vi "RemoteVI Service Client.vi"(0 "Client":T2, 1 "windows":T3(array[cluster]), 5 "geo":T4, 7 "hWnd":u64, 9 "popups":T1, 11 "error in":errorcluster) -> (4 "Client out":T2, 6 "clicked?":bool, 8 "popups out":T1, 15 "error out":errorcluster)   [LabVIEW 2020, in "RemoteVI.lvlib"]
doc: "Services one WebSocket client without blocking (docs\\protocol.md sections 4-6). Reads whatever bytes are waiting (TCP Read, immediate mode, timeout 0; error 56 means nothing waiting, any other error means the peer is gone and sets closed), appends them to rx buffer and decodes every complete frame with RemoteVI WS Decode Client Frame.vi. A text frame goes through RemoteVI Parse Input.vi: an ack raises acked to max(acked, seq) when seq is not ahead of the client's seq; mouse and key messages first update mods (RemoteVI Track Modifiers.vi) and, when they changed and no popup is open, write them into the key state of LabVIEW's UI thread (RemoteVI Apply Modifiers.vi - LabVIEW reads Shift/Ctrl/Alt with GetKeyState, which posted messages do not update), then are translated (RemoteVI Translate Input.vi with geo, popup = popups.windows not empty, and tracking in = LabVIEW holds the mouse capture, RemoteVI Mouse Captured.vi) and posted to the window hWnd (RemoteVI Post Input.vi, which - while a popup is open - moves the invisible popups so that the clicked point lies under the host cursor, never moving the cursor, and waits until the popups change, at most 300 ms; the displacement it used travels on to the next message and out in popups out); a minimized panel is restored first (RemoteVI Restore If Minimized.vi). No VI Server call, so servicing goes on while an open LabVIEW popup blocks the UI thread; the server loop supplies geo, hWnd and popups from its cache. clicked? tells the server loop that a message which may open a LabVIEW popup (anything but WM_MOUSEMOVE and WM_MOUSEWHEEL) was posted, so it holds its VI Server calls back until the popup has had time to appear. A ping is answered with a pong; a close frame with a close frame (1000); a binary or fragmented message with close 1008; a protocol violation with the decoder's close code - each sets closed. Consumed bytes leave rx buffer. A click on a popup is posted no sooner than 350 ms after the popup was first seen open (popup since): LabVIEW ignores a click on a ring menu that arrives within about 250 ms of opening it (measured with posted messages: 200 ms ignored, 250 ms chosen). A client that closes with modifiers written is released (mods set back to 0, unless a popup is open). Mouse and key messages go to the window RemoteVI Route Input.vi picks among windows (docs\\protocol.md section 7); key window - the window the client last pressed a button in - travels from message to message. A client already closed is passed through untouched. TCP errors only set closed; error out carries the errors of restoring the window and posting input."
uses:
  RemoteVI.lvlib
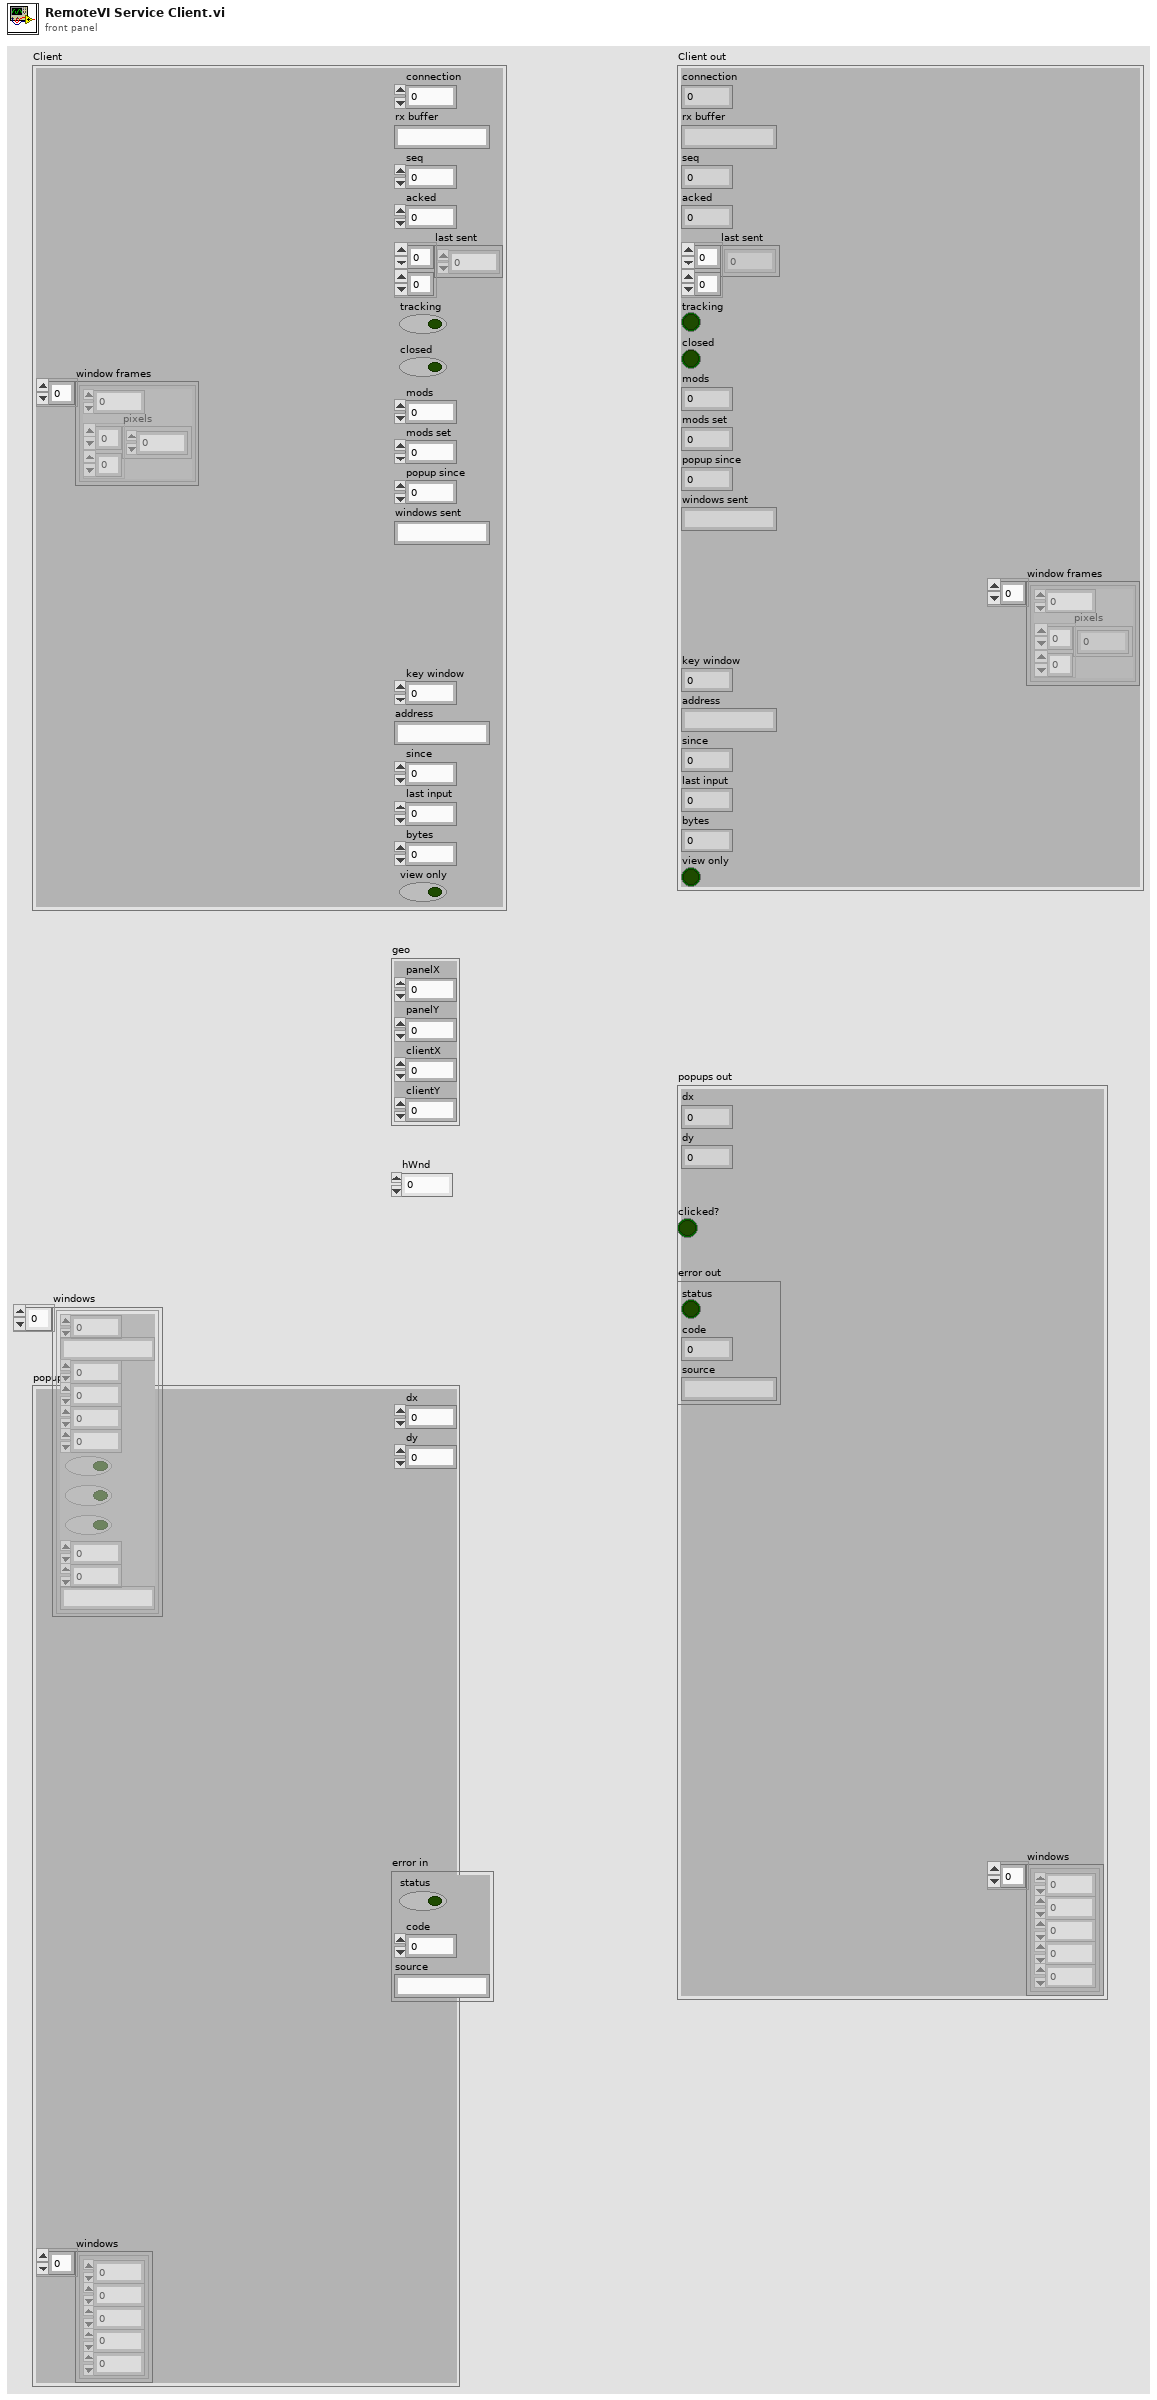
[diagram p1: front panel]
types:
  T1 = cluster{"windows":cluster{"hwnd":u64, "x":i32, "y":i32, "w":i32, "h":i32}[], "dx":i32, "dy":i32}
  T2 = cluster{"connection":u32, "rx buffer":string, "seq":u32, "acked":u32, "last sent":u32[][], "tracking":bool, "closed":bool, "mods":u8, "mods set":u8, "popup since":u32, "windows sent":string, "window frames":cluster{"id":u64, "pixels":u32[][]}[], "key window":u64, "address":string, "since":dbl, "last input":dbl, "bytes":dbl, "view only":bool}
  T3 = cluster{"id":u64, "title":string, "x":i32, "y":i32, "w":i32, "h":i32, "modal":bool, "active":bool, "closable":bool, "sx":i32, "sy":i32, "class":string}[]
  T4 = cluster{"panelX":i32, "panelY":i32, "clientX":i32, "clientY":i32}
  T5 = cluster{"hWnd":u64, "popup":bool, "geo":cluster{"panelX":i32, "panelY":i32, "clientX":i32, "clientY":i32}}
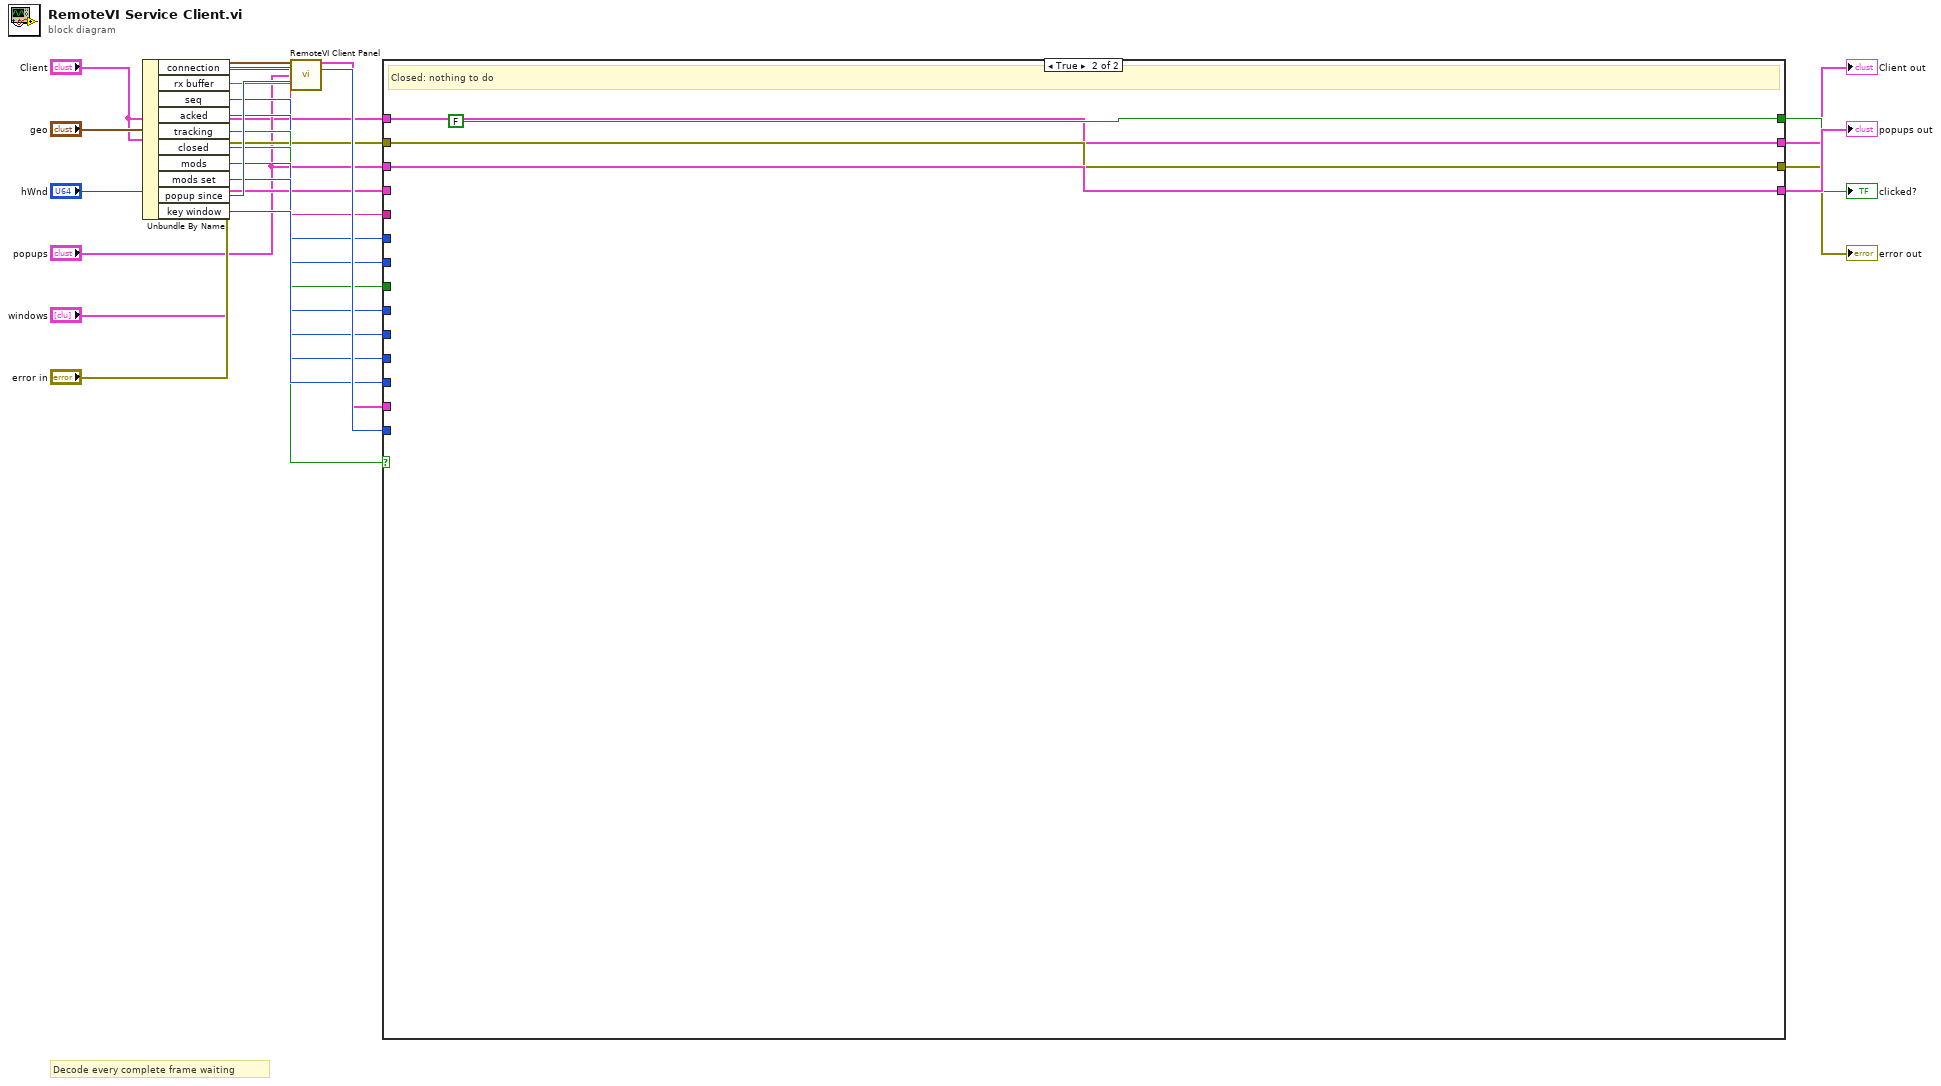
[diagram p0: block diagram]
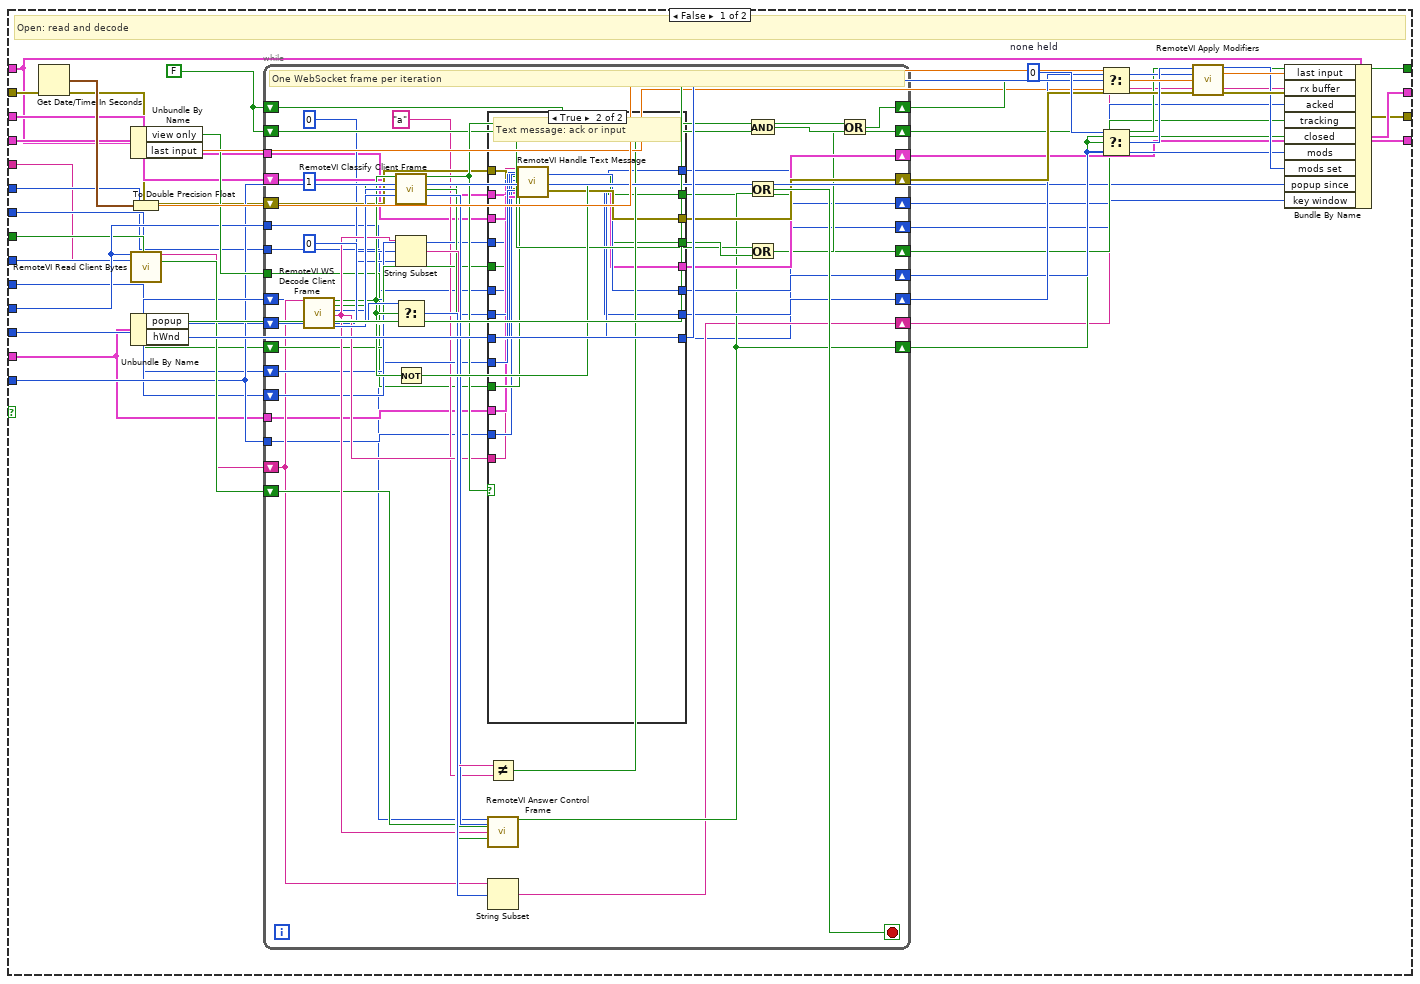
[diagram p2: hidden frame]
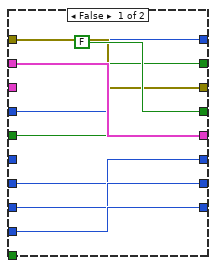
[diagram p3: hidden frame]
diagram:
  # "Decode every complete frame waiting"
  n1 = Unbundle By Name("Client") -> ("connection"=w7:u32, "rx buffer"=w8:string, "seq"=w9:u32, "acked"=w10:u32, "tracking"=w11:bool, "closed"=w12:bool, "mods"=w13:u8, "mods set"=w14:u8, "popup since"=w15:u32, "key window"=w16:u64)
  n2 = call "RemoteVI Client Panel.vi"("geo"="geo", "hWnd"="hWnd", "popups"="popups", "popup since"=w15) -> ("panel"=w17:T5, "popup since out"=w18:u32)  [unwired: 10 in]
  n3 = case shown="True" w12 {
    tunnel: "Client" -> [w23 w141]
    tunnel: "error in" -> [w24 w142]
    tunnel: "popups" -> [w30 w143]
    tunnel: "windows" -> [w35 _]
    tunnel: [w48 FALSE] -> w21
    tunnel: w8 -> [w25 _]
    tunnel: w9 -> [w26 _]
    tunnel: w10 -> [w27 _]
    tunnel: w11 -> [w28 _]
    tunnel: w13 -> [w31 _]
    tunnel: w14 -> [w32 _]
    tunnel: w7 -> [w34 _]
    tunnel: w16 -> [w36 _]
    tunnel: [w62 w141] -> w19
    tunnel: [w58 w142] -> w20
    tunnel: [w49 w143] -> w22
    tunnel: w17 -> [w29 _]
    tunnel: w18 -> [w33 _]
    frame False {
      w55 = u8 0  # none held
      w39 = FALSE
      # "Open: read and decode"
      n4 = Get Date/Time In Seconds() -> (seconds since 1Jan1904=w59:timestamp)
      n5 = Unbundle By Name(w23) -> ("view only"=w40:bool, "last input"=w41:dbl)
      n6 = To Double Precision Float(number=w59) -> (double precision float=w60:dbl)
      n7 = call "RemoteVI Read Client Bytes.vi"("connection"=w34, "rx buffer"=w25) -> ("rx buffer out"=w37:string, "gone?"=w38:bool)  [unwired: 12 in]
      n8 = Unbundle By Name(w29) -> ("popup"=w53:bool, "hWnd"=w54:u64)
      n9 = while {
        shift-right: [w70] -> w42
        shift-left: w39 -> [w69]
        shift-right: [w85] -> w48
        shift-left: w39 -> [w84]
        tunnel: w35 -> [w67]
        shift-right: [w88] -> w49
        shift-left: w30 -> [w87]
        shift-right: [w94] -> w52
        shift-left: w24 -> [w93]
        tunnel: w34 -> [w63]
        tunnel: w26 -> [w64]
        tunnel: w40 -> [w68]
        shift-right: [w75] -> w43
        shift-left: w36 -> [w74]
        shift-right: [w79] -> w45
        shift-left: w27 -> [w78]
        shift-right: [w81] -> w46
        shift-left: w28 -> [w80]
        shift-right: [w90] -> w50
        shift-left: w31 -> [w89]
        shift-right: [w92] -> w51
        shift-left: w32 -> [w91]
        tunnel: w29 -> [w65]
        tunnel: w33 -> [w66]
        shift-right: [w77] -> w44
        shift-left: w37 -> [w76]
        shift-right: [w83] -> w47
        shift-left: w38 -> [w82]
        stop <- w111 stop-if-true
        # "One WebSocket frame per iteration"
        n10 = call "RemoteVI WS Decode Client Frame.vi"("buffer"=w76) -> ("complete?"=w95:bool, "fin"=w96:bool, "opcode"=w97:u8, "payload"=w98:string, "bytes consumed"=w99:u32, "close code"=w100:u16)  [unwired: 13 in]
        n11 = call "RemoteVI Classify Client Frame.vi"("complete?"=w95, "fin"=w96, "opcode"=w97, "close code"=w100) -> ("text?"=w101:bool, "ping?"=w102:bool, "close?"=w103:bool, "close code out"=w104:u16)  [unwired: 8 in]
        n12 = String Subset(string=w98, offset (0)=0, length (rest)=1) -> (substring=w105:string)
        n13 = Select(t=w99, s=w95, f=u32 0) -> (s? t:f=w109:u32)
        n14 = Not(x=w95) -> (.not. x?=w110:bool)
        n15 = case shown="True" w101 {
          tunnel: w93 -> [w114 w123]
          tunnel: w87 -> [w115 w126]
          tunnel: w67 -> [_ w130]
          tunnel: w78 -> [w112 w121]
          tunnel: w80 -> [w113 w122]
          tunnel: w64 -> [_ w124]
          tunnel: w89 -> [w116 w127]
          tunnel: w91 -> [w117 w128]
          tunnel: w74 -> [w118 w131]
          tunnel: w68 -> [_ w132]
          tunnel: w65 -> [_ w125]
          tunnel: w66 -> [_ w129]
          tunnel: w98 -> [_ w120]
          tunnel: [w112 w133] -> w79
          tunnel: [w113 w134] -> w81
          tunnel: [w114 w140] -> w94
          tunnel: [FALSE w135] -> w86
          tunnel: [w115 w136] -> w88
          tunnel: [w116 w137] -> w90
          tunnel: [w117 w138] -> w92
          tunnel: [w118 w139] -> w75
          frame False {
          }
          frame True {
            # "Text message: ack or input"
            n16 = call "RemoteVI Handle Text Message.vi"("text"=w120, "acked"=w121, "tracking"=w122, "seq"=w124, "panel"=w125, "error in"=w123, "popups"=w126, "windows"=w130, "mods"=w127, "key window"=w131, "mods set"=w128, "popup since"=w129, "view only?"=w132) -> ("mods set out"=w138:u8, "key window out"=w139:u64, "acked out"=w133:u32, "tracking out"=w134:bool, "clicked?"=w135:bool, "popups out"=w136:T1, "mods out"=w137:u8, "error out"=w140:errorcluster)  [unwired: 7 in]
          }
        }
        n17 = Not Equal?(x=w105, y="a") -> (x != y?=w106:bool)
        n18 = call "RemoteVI Answer Control Frame.vi"("connection"=w63, "close code"=w104, "closed?"=w82, "ping?"=w102, "payload"=w98, "close?"=w103) -> ("closed out"=w83:bool)  [unwired: 9 in]
        n19 = String Subset(string=w76, offset (0)=w109) -> (substring=w77:string)  [unwired: 1 in]
        n20 = And(x=w101, y=w106) -> (x .and. y?=w107:bool)
        n21 = Or(x=w110, y=w83) -> (x .or. y?=w111:bool)
        n22 = Or(x=w84, y=w86) -> (x .or. y?=w85:bool)
        n23 = Or(x=w69, y=w107) -> (x .or. y?=w70:bool)
      }
      n24 = Select(t=w60, s=w42, f=w41) -> (s? t:f=w61:dbl)
      n25 = Select(t=w55, s=w47, f=w50) -> (s? t:f=w56:u8)
      n26 = call "RemoteVI Apply Modifiers.vi"("mods"=w56, "mods set"=w51, "popup"=w53, "hWnd"=w54, "error in"=w52) -> ("mods set out"=w57:u8, "error out"=w58:errorcluster)  [unwired: 9 in]
      n27 = Bundle By Name(cluster=w23, "last input"=w61, "rx buffer"=w44, "acked"=w45, "tracking"=w46, "closed"=w47, "mods"=w50, "mods set"=w57, "popup since"=w33, "key window"=w43) -> (w62:T2)
    }
    frame True {
      # "Closed: nothing to do"
    }
  }
  "Client out" <- w19
  "popups out" <- w22
  "clicked?" <- w21
  "error out" <- w20
